vi "VHistFile - Build Path in App directory.vi"(4 "path in":path) -> (1 "path out":path)   [LabVIEW 2021]
doc: "The VI transforms a relative path to an absolute path in relation to a directory where the top-level VI in its call chain resides. If an input path is empty, the VI returns a directory path of the top-level VI. If an input path is either an absolute path or <Not A Path>, VI returns the same value as an input.\n\n::: CalcExpress Toolkit :::\nCopyright (c) 2000-2026 Konstantin Shifershteyn. All rights reserved."
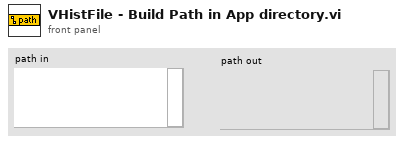
[diagram p1: front panel]
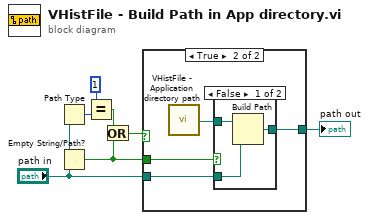
[diagram p0: block diagram]
diagram:
  n1 = Path Type(1:"path in") -> (0:w5:i16)
  n2 = Empty String/Path?(string/path="path in") -> (empty?=w1:bool)
  n3 = Equal?(x=i16 1, y=w5) -> (x = y?=w3:bool)
  n4 = Or(x=w3, y=w1) -> (x .or. y?=w2:bool)
  n5 = case shown="True" w2 {
    tunnel: "path in" -> [w8 w12]
    tunnel: [w8 w11] -> w7
    tunnel: w1 -> [_ w10]
    frame False {
    }
    frame True {
      n6 = call "VHistFile - Application directory path.vi"() -> ("application directory path"=w9:path)
      n7 = case shown="False" w10 {
        tunnel: w9 -> [w15 w16]
        tunnel: w12 -> [w14 _]
        tunnel: [w13 w16] -> w11
        frame False {
          n8 = Build Path(base path=w15, name or relative path=w14) -> (appended path=w13:path)
        }
        frame True {
        }
      }
    }
  }
  "path out" <- w7
